vi "destroy batch buffer.vi"(11 "batch buffer":refnum<data-value>) -> (0 "error out":errorcluster)   [LabVIEW 2020, in "nominal core steps.lvlib"]
doc: "Immediately destroy the buffer. Does not flush."
uses:
  nominal core steps.lvlib
  batch buffer.ctl
  channel uid.ctl
  points buffer.ctl
  single point.ctl
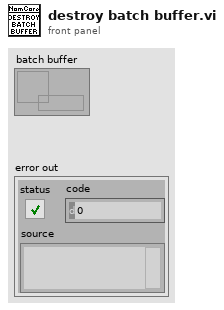
[diagram p1: front panel]
types:
  T1 = typedef "nominal core steps.lvlib/batch buffer.ctl" = map{T2, refnum<data-value>}
  T2 = typedef "nominal core steps.lvlib/channel uid.ctl" = cluster{"channel name":string, "tags":map{string, string}}
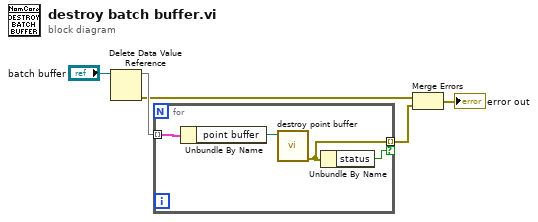
[diagram p0: block diagram]
diagram:
  n1 = Delete Data Value Reference(data value reference="batch buffer") -> (data value=w4:T1, error out=w2:errorcluster)  [unwired: 1 in]
  n2 = for {
    tunnel: w4 -> [w9] mode=indexing
    tunnel: [w7] -> w1 mode=indexing if=w6
    n3 = Unbundle By Name(w9) -> ("point buffer"=w8:refnum<data-value>)
    n4 = call "destroy point buffer.vi"("point buffer"=w8) -> ("error out"=w7:errorcluster)  [unwired: 10 in]
    n5 = Unbundle By Name(w7) -> ("status"=w6:bool)
  }
  n6 = Merge Errors(w2, w1) -> (→"error out":errorcluster)
